vi "TEMPLATE.vi"(6 "Teller":refnum<class "Teller.lvclass">, 8 "Error in":errorcluster, 11 "TEMPLATE jettl Msg in":refnum<class "TEMPLATE jettl Msg.lvclass">) -> (0 "Error out":errorcluster, 3 "TEMPLATE jettl Msg out":refnum<class "TEMPLATE jettl Msg.lvclass">)   [LabVIEW 2020, in "_Template.lvlib" / "Templates.lvlib" / "TEMPLATE jettl Msg.lvlib" / "TEMPLATE jettl Msg.lvclass"]
uses:
  TEMPLATE jettl Msg.lvclass
  jettl/jettl/Teller/Teller.lvclass
panel:
  # "Optionally add controls to the front panel and wire to connector pane terminal postions 10 and/or 9 (the two left middle terminals for the 4x2x2x4 conn pane).\n\nOptionally add indicators to the front panel and wire to connector pane terminal postions 2 and/or 1 (the two right middle terminals for the 4x2x2x4 conn pane)."
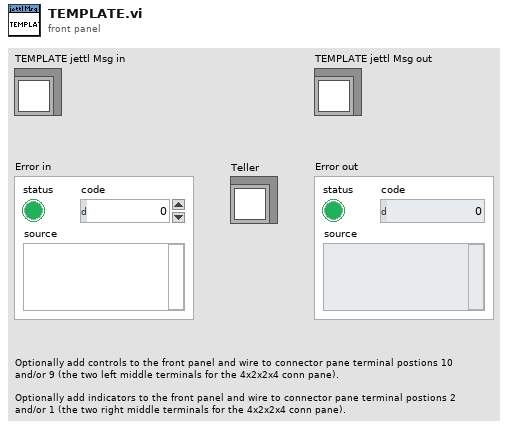
[diagram p1: front panel]
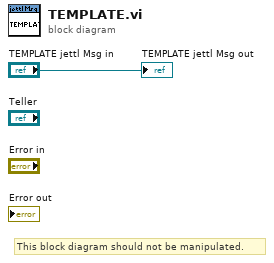
[diagram p0: block diagram]
diagram:
  # "This block diagram should not be manipulated."
  "TEMPLATE jettl Msg out" <- "TEMPLATE jettl Msg in"
